vi "simple test API.vi"() -> ()   [LabVIEW 2013]
uses:
  dynamic profibus/full response.ctl
  dynamic profibus/profibus master transmit header.ctl
  dynamic profibus/full command.ctl
  dynamic profibus/profibus master action.ctl
  <vilib>/Utility/RT CPU Load.ctl
  <vilib>/Utility/RT CPU pool selections.ctl
  <vilib>/Platform/TimedLoop/XDataNode/timing_clust.ctl
  <vilib>/Platform/TimedLoop/XDataNode/nitl_modes.ctl
  <vilib>/Platform/TimedLoop/XDataNode/wakeup.ctl
  dynamic profibus/parse response value.vi
  <vilib>/FPGAPlugInAG/cRIO-9068/niLvFpga_Open_cRIO-9068.vi
  <vilib>/rvi/interface/common/dynamic/niFpgaDynamicAddResources.vi
  <vilib>/FPGAPlugInAG/Dynamic/niLvFpga_Reset_Dynamic.vi
  <vilib>/FPGAPlugInAG/Dynamic/niLvFpga_Run_Dynamic.vi
  dynamic profibus/read raw commands.vi
  <vilib>/FPGAPlugInAG/Dynamic/niLvFpga_Close_Dynamic.vi
  <vilib>/platform/TimedLoop/XDataNode/XDataNode.xnode
  <vilib>/rvi/interface/nirviOpenFPGA/nirviOpenFPGA.xnode
  FPGA Bitfiles/ProfibusModule_FPGATargetMSlave_FPGAMain_hsONVj+8C84.lvbitx
  execution/FPGA Main.vi
  <vilib>/rvi/interface/nirviMethod/nirviMethod.xnode
  <vilib>/rvi/interface/nirviCloseFPGA/nirviCloseFPGA.xnode
  dynamic profibus/dynamic profibus.lvlib
  <vilib>/NI_Real-Time Target Support.lvlib
  <vilib>/Platform/TimedLoop/XDataNode/XDNodeRunTimeDep.lvlib
panel:
  out "Empty Elements Remaining":u32
  in  "sending":bool
  in  "set":bool
  in  "stop cpu":bool
  out "CPU loads":T1[](array[typedef]) {"ISR (%)" format="%#.2f"; "Idle (%)" format="%#.2f"; "Background (%)" format="%#.2f"; "Normal (%)" format="%#.2f"; "Above Normal (%)" format="%#.2f"; "High (%)" format="%#.2g"; "Timed Structures (%)" format="%#.2g"; "Time Critical (%)" format="%#.2g"; "Total (%)" format="%#.2g"}
  out "Numeric":i32
  in  "milliseconds to wait":u32=100
  in  "stop":bool
  in  "commands":T2[](array[typedef])=[{"action"=enum."get input", "device"=0, "index"=1, "data"=0}, {"action"=enum."set output", "device"=0, "index"=5, "data"=2}, {"action"=enum."transfer data", "device"=0, "index"=3, "data"=0}, {"action"=enum."get input", "device"=0, "index"=4, "data"=0}]
  out "responses":T4[](array[typedef])
  out "Slave Info List":T6(array[cluster])
  out "error out":errorcluster
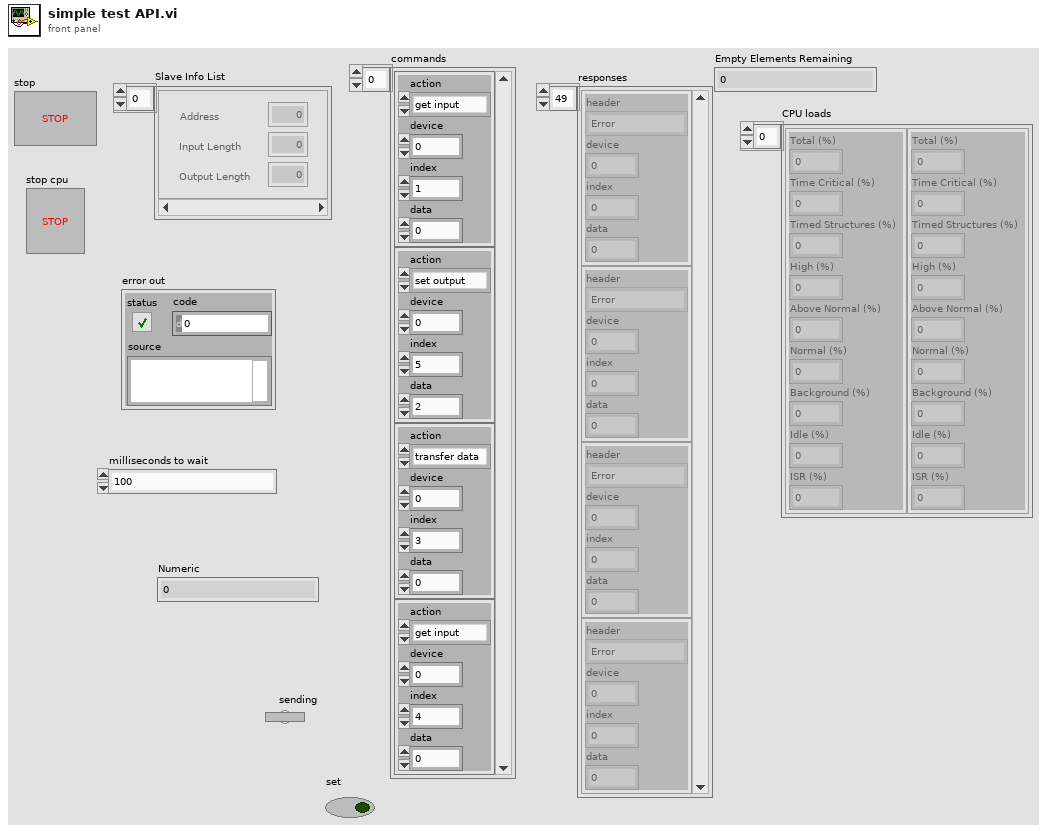
[diagram p1: front panel]
types:
  T1 = typedef "NI_Real-Time Target Support.lvlib/RT CPU Load.ctl" = cluster{"Total (%)":dbl, "Time Critical (%)":dbl, "Timed Structures (%)":dbl, "High (%)":dbl, "Above Normal (%)":dbl, "Normal (%)":dbl, "Background (%)":dbl, "Idle (%)":dbl, "ISR (%)":dbl}
  T2 = typedef "dynamic profibus.lvlib/full command.ctl" = cluster{"action":T3, "device":u8, "index":u8, "data":u8}
  T3 = typedef "dynamic profibus.lvlib/profibus master action.ctl" = enum8{"initialize", "uninitialize", "stop", "get input", "get input size", "set output", "get output size", "get diagnostic", "transfer data", "transfer diagnostics", "read many inputs"}
  T4 = typedef "dynamic profibus.lvlib/full response.ctl" = cluster{"header":T5, "device":u8, "index":u8, "data":u8}
  T5 = typedef "dynamic profibus.lvlib/profibus master transmit header.ctl" = enum8{"Error", "Input", "Diagnostic", "input size", "output size", "many inputs"}
  T6 = cluster{"Address":i8, "Input Length":u8, "Output Length":u8}[]
  T7 = typedef "NI_Real-Time Target Support.lvlib/RT CPU pool selections.ctl" = enum16{"System & Timed Structures", "System", "Timed Structures", "Reserved"}
  T8 = typedef "XDNodeRunTimeDep.lvlib/timing_clust.ctl" = cluster{"Expected End [f-1]":u64, "Actual End [f-1]":u64, "Finished Late? [f-1]":bool, "Expected End [i-1]":u64, "Actual End [i-1]":u64, "Finished Late? [i-1]":bool, "Expected Start [i]":u64, "Actual Start [i]":u64, "Expected Start [f]":u64, "Actual Start [f]":u64, "Source Name":string, "Structure Name":string, "Period":i64, "Deadline":i64, "Offset":i64, "Start":i64, "Priority":i32, "Timeout":i32, "Mode":T9, "Wakeup Reason":T10, "Error":errorcluster, "Source Type":string, "Secondary Source Type":string, "Global End Time":u64, "Global Start Time":u64, "Frame Duration":u64, "Iteration Duration":u64, "Assigned CPU":i32, "I/O Scan Engine Mode":u32}
  T9 = typedef "XDNodeRunTimeDep.lvlib/nitl_modes.ctl" = enum32{"No Change", "Process missed periods, maintain original phase", "Discard missed periods, maintain original phase", "Process missed periods, ignore original phase", "Discard missed periods, ignore original phase"}
  T10 = typedef "XDNodeRunTimeDep.lvlib/wakeup.ctl" = enum32{"Normal", "Aborted", "Asynchronous wakeup", "Timing source error", "Timed loop error", "Timeout"}
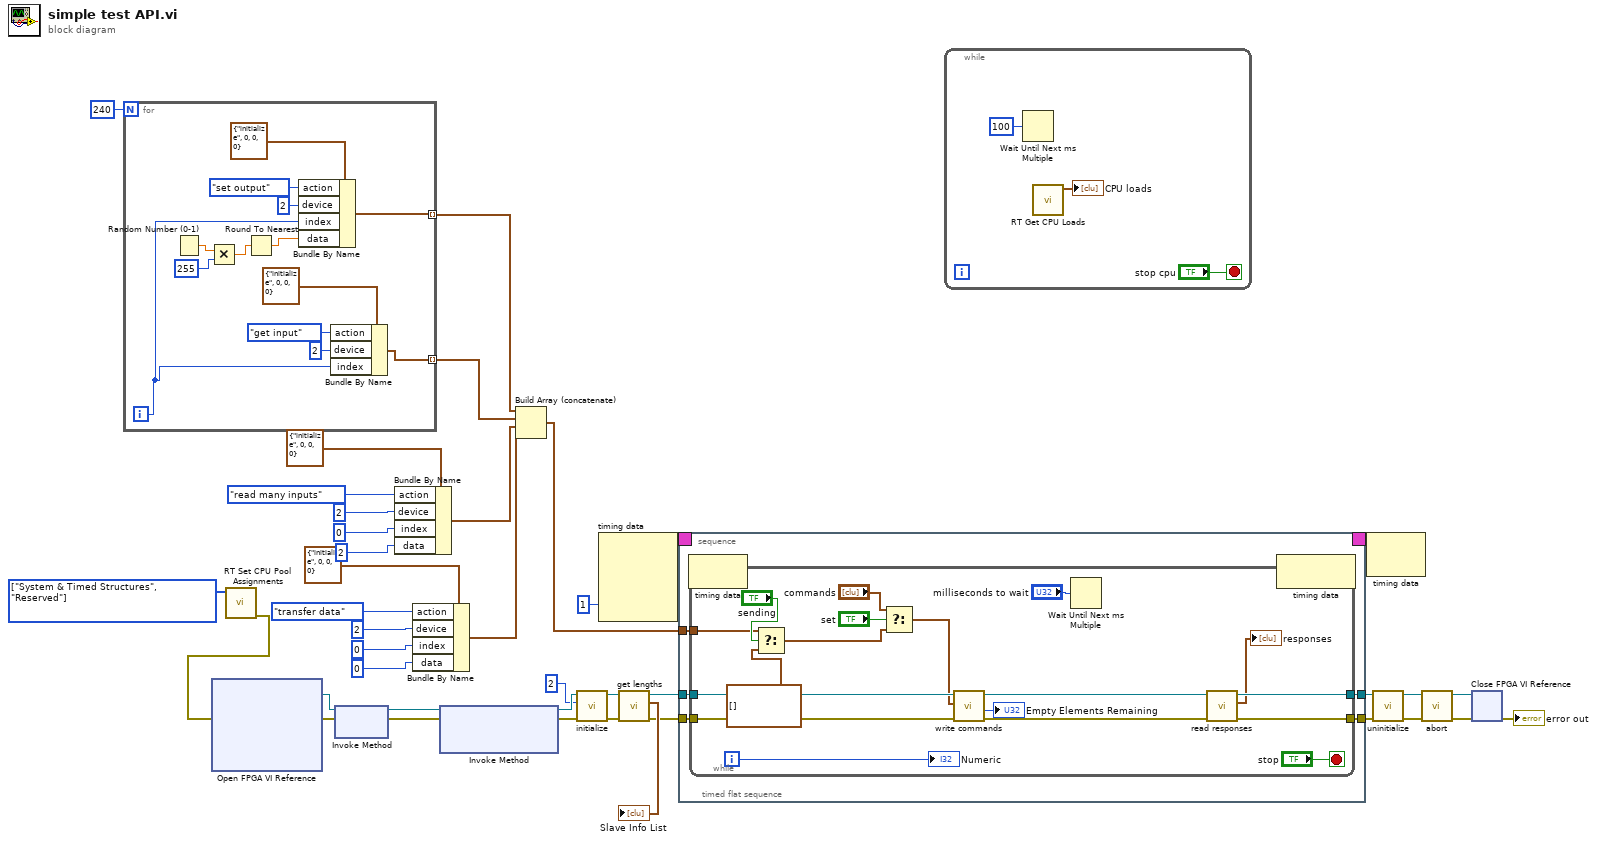
[diagram p0: block diagram]
diagram:
  w20 = T7[] [enum."System & Timed Structures", enum."Reserved"] items=["System & Timed Structures", "System", "Timed Structures", "Reserved"] ("CPU pools")
  n1 = for {
    N: 240 -> [_]
    tunnel: [w50] -> w9 mode=indexing
    tunnel: [w42] -> w7 mode=indexing
    i -> [w41]
    n2 = Random Number (0-1)() -> (number: 0 to 1=w49:dbl)
    n3 = Multiply(x=w49, y=u8 255 ("data")) -> (x*y=w47:dbl)
    n4 = Round To Nearest(number=w47) -> (nearest integer value=w46:dbl)
    n5 = Bundle By Name(cluster=T2 {"action"=enum."initialize", "device"=0, "index"=0, "data"=0} ("command"), "action"=profibus_master_action."set output", "device"=u8 2, "index"=w41, "data"=w46) -> (w50:T2)
    n6 = Bundle By Name(cluster=T2 {"action"=enum."initialize", "device"=0, "index"=0, "data"=0} ("command"), "action"=profibus_master_action."get input", "device"=u8 2, "index"=w41) -> (w42:T2)
  }
  n7 = call <vilib>:"RT Set CPU Pool Assignments.vi"("CPU pools"=w20) -> ("error out"=w21:errorcluster)  [unwired: 7 in, 3 out]
  n8 = xnode "Open FPGA VI Reference"("error in"=w21) -> ("FPGA VI Reference Out"=w36:refnum<k20>, "error out"=w38:errorcluster)  [unwired: 1 in]
  n9 = xnode "Invoke Method"("FPGA VI Reference In"=w36, "error in"=w38) -> ("FPGA VI Reference Out"=w34:refnum<k20>, "error out"=w37:errorcluster)
  n10 = Bundle By Name(cluster=T2 {"action"=enum."initialize", "device"=0, "index"=0, "data"=0} ("command"), "action"=profibus_master_action."read many inputs", "device"=u8 2, "index"=u8 0, "data"=u8 2) -> (w1:T2)
  n11 = Bundle By Name(cluster=T2 {"action"=enum."initialize", "device"=0, "index"=0, "data"=0} ("command"), "action"=profibus_master_action."transfer data", "device"=u8 2, "index"=u8 0, "data"=u8 0) -> (w10:T2)
  n12 = xnode "Invoke Method"("FPGA VI Reference In"=w34, "error in"=w37) -> ("FPGA VI Reference Out"=w33:refnum<k20>, "error out"=w35:errorcluster)  [unwired: 1 in]
  n13 = Build Array (concatenate)(w9, w7, w1, w10) -> (w8:T2[])
  n14 = call "initialize.vi"("error in"=w35, "device (if slave)"=u8 2, "profibus reference"=w33) -> ("error out"=w40:errorcluster, "profibus reference out"=w39:refnum<k20>)  [unwired: 7 in]
  n15 = node-c288(1 ("Processor")) -> (w19:T8)  [unwired: 3 in]
  n16 = call "get lengths.vi"("error in"=w40, "profibus reference"=w39) -> ("error out"=w25:errorcluster, "Slave Info List"=→"Slave Info List":T6, "profibus reference out"=w26:refnum<k20>)  [unwired: 7 in]
  n17 = timed-sequence {
    timing: w19 -> [_]
    timing-out: [_] -> w18
    tunnel: w26 -> [w58]
    tunnel: w25 -> [w57]
    tunnel: [w56] -> w24
    tunnel: [w55] -> w23
    tunnel: w8 -> [w54]
    n18 = timed-flat-sequence {
      tunnel: w58 -> [w63]
      tunnel: w57 -> [w62]
      tunnel: [w61] -> w56
      tunnel: [w60] -> w55
      tunnel: w54 -> [w59]
      n19 = node-c288() -> ()  [unwired: 1 in, 1 out]
      n20 = while {
        tunnel: w63 -> [w81]
        tunnel: w62 -> [w80]
        tunnel: [w79] -> w61
        tunnel: [w78] -> w60
        tunnel: w59 -> [w66]
        i -> [w73]
        stop <- "stop" stop-if-true
        n21 = Select(t=w66, s="sending", f=T2[] [] ("commands 2")) -> (s? t:f=w67:T2[])
        n22 = Select(t="commands", s="set", f=w67) -> (s? t:f=w70:T2[])
        n23 = call "write commands.vi"("error in"=w80, "commands"=w70, "profibus reference"=w81) -> ("error out"=w76:errorcluster, "Empty Elements Remaining"=→"Empty Elements Remaining":u32, "profibus reference out"=w77:refnum<k20>)  [unwired: 6 in]
        n24 = Wait Until Next ms Multiple(millisecond multiple="milliseconds to wait") -> ()  [unwired: 1 out]
        n25 = call "read responses.vi"("error in"=w76, "profibus reference"=w77) -> ("error out"=w78:errorcluster, "responses"=→"responses":T4[], "profibus reference out"=w79:refnum<k20>)  [unwired: 7 in]
        "Numeric" <- w73
      }
      n26 = node-c288() -> ()  [unwired: 1 in, 1 out]
    }
  }
  n27 = while {
    stop <- "stop cpu" stop-if-true
    n28 = Wait Until Next ms Multiple(millisecond multiple=u32 100) -> ()  [unwired: 1 out]
    n29 = call <vilib>:"RT Get CPU Loads.vi"() -> ("CPU loads"=→"CPU loads":T1[])  [unwired: 10 in, 1 out]
  }
  n30 = node-c288(w18) -> ()  [unwired: 1 out]
  n31 = call "uninitialize.vi"("error in"=w23, "profibus reference"=w24) -> ("error out"=w31:errorcluster, "profibus reference out"=w32:refnum<k20>)  [unwired: 8 in]
  n32 = call "abort.vi"("error in"=w31, "profibus reference"=w32) -> ("error out"=w29:errorcluster, "profibus reference out"=w30:refnum<k20>)  [unwired: 8 in]
  n33 = xnode "Close FPGA VI Reference"("FPGA VI Reference In"=w30, "error in"=w29) -> ("error out"=→"error out":errorcluster)
